vi "test modern initialize.vi"(8 "error in (no error)":errorcluster) -> (0 "error out":errorcluster, 3 "body":string)   [LabVIEW 2020, in "MCP Server tests.lvlib"]
doc: "initialize does not exist in the modern era (MCP 2026-07-28). Sent with the modern headers and a complete params._meta it is answered HTTP 404 with the JSON-RPC error -32601 and the request id. A legacy initialize (no MCP-Protocol-Version header, no _meta) is still answered 200 with result.protocolVersion. The requests are sent with the LabVIEW HTTP Client directly."
uses:
  MCP Server tests.lvlib
  <vilib>/addons/_JKI Toolkits/Caraya/classes/Test/Test.lvclass
  <vilib>/addons/_JKI Toolkits/Caraya/classes/Assert/Assert.lvclass
panel:
  out "lookup error":errorcluster
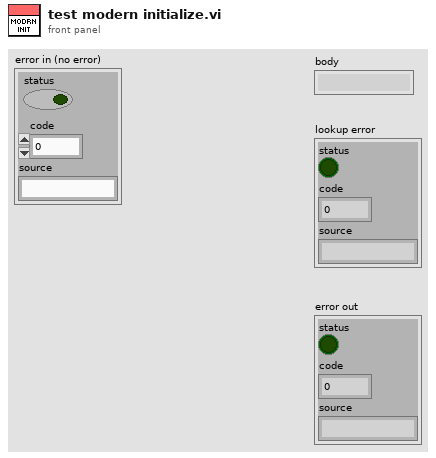
[diagram p1: front panel]
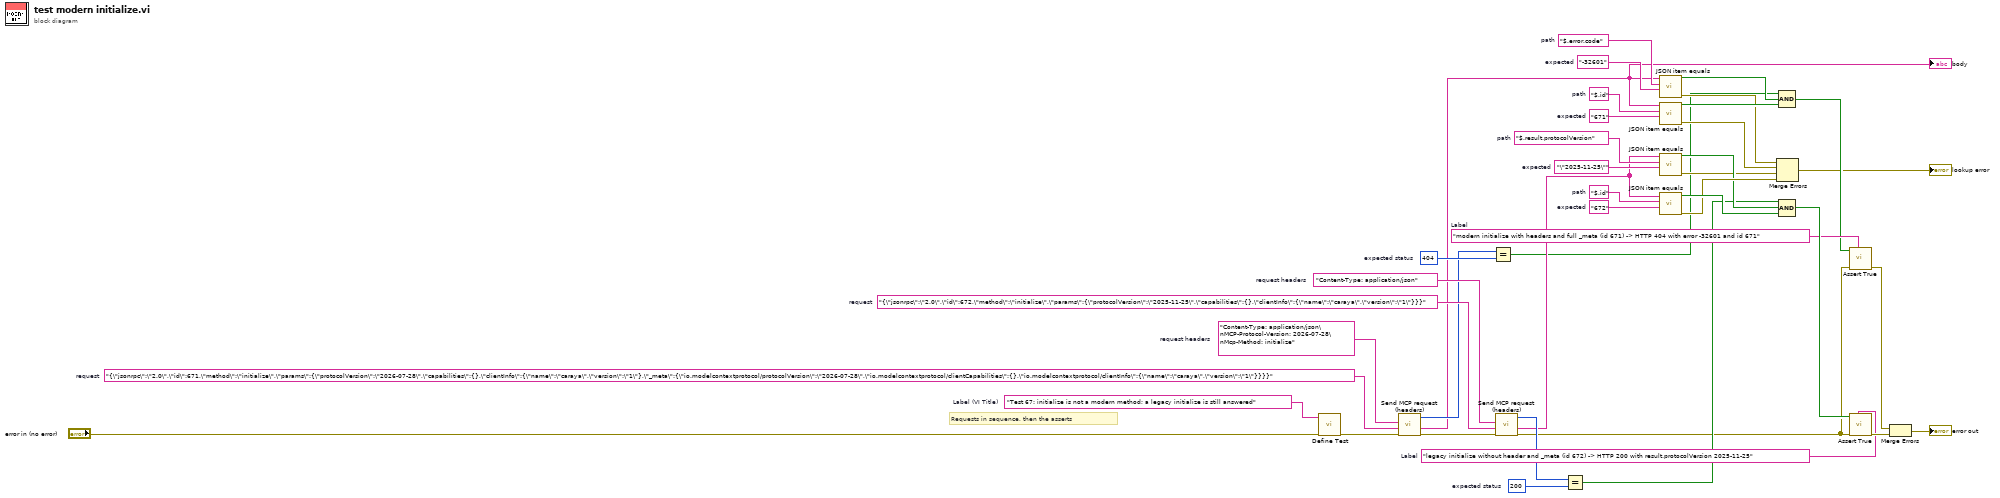
[diagram p0: block diagram]
diagram:
  w39 = "legacy initialize without header and _meta (id 672) -> HTTP 200 with result.protocolVersion 2025-11-25"  # Label
  w36 = "modern initialize with headers and full _meta (id 671) -> HTTP 404 with error -32601 and id 671"  # Label
  w31 = "672"  # expected
  w30 = "$.id"  # path
  w27 = "\"2025-11-25\""  # expected
  w26 = "$.result.protocolVersion"  # path
  w24 = 200  # expected status
  w20 = "Content-Type: application/json"  # request headers
  w19 = "{\"jsonrpc\":\"2.0\",\"id\":672,\"method\":\"initialize\",\"params\":{\"protocolVersion\":\"2025-11-25\",\"capabilities\":{},\"clientInfo\":{\"name\":\"caraya\",\"version\":\"1\"}}}"  # request
  w16 = "671"  # expected
  w15 = "$.id"  # path
  w12 = "-32601"  # expected
  w11 = "$.error.code"  # path
  w9 = 404  # expected status
  w5 = "Content-Type: application/json\nMCP-Protocol-Version: 2026-07-28\nMcp-Method: initialize"  # request headers
  w4 = "{\"jsonrpc\":\"2.0\",\"id\":671,\"method\":\"initialize\",\"params\":{\"protocolVersion\":\"2026-07-28\",\"capabilities\":{},\"clientInfo\":{\"name\":\"caraya\",\"version\":\"1\"},\"_meta\":{\"io.modelcontextprotocol/protocolVersion\":\"2026-07-28\",\"io.modelcontextprotocol/clientCapabilities\":{},\"io.modelcontextprotocol/clientInfo\":{\"name\":\"caraya\",\"version\":\"1\"}}}}"  # request
  w2 = "Test 67: initialize is not a modern method; a legacy initialize is still answered"  # Label (VI Title)
  # "Requests in sequence, then the asserts"
  n1 = call <vilib>:"Define Test.vi"("error in (no error)"="error in (no error)", "Label (VI Title)"=w2) -> ("error out"=w3:errorcluster)  [unwired: 8 in, 1 out]
  n2 = call "Send MCP request (headers).vi"("error in (no error)"=w3, "request"=w4, "request headers"=w5) -> ("error out"=w6:errorcluster, "response"=w7:string, "status code"=w8:i32)  [unwired: 5 in, 1 out]
  "body" <- w7
  n3 = Equal?(x=w8, y=w9) -> (x = y?=w10:bool)
  n4 = call "Send MCP request (headers).vi"("error in (no error)"=w6, "request"=w19, "request headers"=w20) -> ("error out"=w21:errorcluster, "response"=w22:string, "status code"=w23:i32)  [unwired: 5 in, 1 out]
  n5 = Equal?(x=w23, y=w24) -> (x = y?=w25:bool)
  n6 = call "JSON item equals.vi"("expected"=w12, "path"=w11, "JSON"=w7) -> ("error out"=w13:errorcluster, "equal?"=w14:bool)  [unwired: 6 in, 1 out]
  n7 = call "JSON item equals.vi"("expected"=w16, "path"=w15, "JSON"=w7) -> ("error out"=w17:errorcluster, "equal?"=w18:bool)  [unwired: 6 in, 1 out]
  n8 = call "JSON item equals.vi"("expected"=w27, "path"=w26, "JSON"=w22) -> ("error out"=w28:errorcluster, "equal?"=w29:bool)  [unwired: 6 in, 1 out]
  n9 = call "JSON item equals.vi"("expected"=w31, "path"=w30, "JSON"=w22) -> ("error out"=w32:errorcluster, "equal?"=w33:bool)  [unwired: 6 in, 1 out]
  n10 = Merge Errors(w13, w17, w28, w32) -> (→"lookup error":errorcluster)
  n11 = Compound Arithmetic op=AND(w10, w14, w18) -> (w35:bool)
  n12 = Compound Arithmetic op=AND(w25, w29, w33) -> (w38:bool)
  n13 = call <vilib>:"Assert True.vi"("Label"=w36, "error in (no error)"=w21, "True?"=w35) -> ("error out"=w37:errorcluster)  [unwired: 7 in, 1 out]
  n14 = call <vilib>:"Assert True.vi"("Label"=w39, "error in (no error)"=w21, "True?"=w38) -> ("error out"=w40:errorcluster)  [unwired: 7 in, 1 out]
  n15 = Merge Errors(w37, w40) -> (→"error out":errorcluster)
